vi "DAQmx.AO Max to Range.vi"(11 "AO.Max":dbl) -> (3 "Range":T1)   [LabVIEW 2019, in "DAQmx.lvclass"]
uses:
  DAQmx.lvclass
  typedefs/DAQmx.Config.AO.Range--enum.ctl
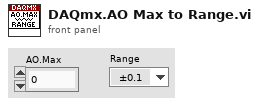
[diagram p1: front panel]
types:
  T1 = typedef "DAQmx.lvclass/DAQmx.Config.AO.Range--enum.ctl" = enum16{"±0.1", "±1.0", "±3.5", "±10.0"}
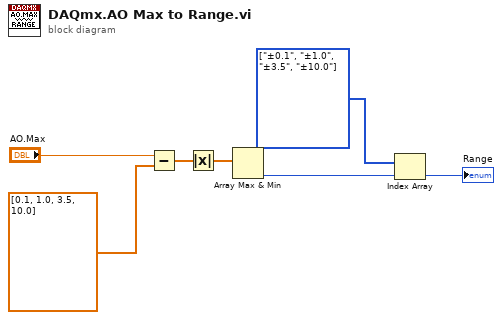
[diagram p0: block diagram]
diagram:
  w3 = T1[] [enum."±0.1", enum."±1.0", enum."±3.5", enum."±10.0"] items=["±0.1", "±1.0", "±3.5", "±10.0"] ("Range")
  n1 = Subtract(x="AO.Max", y=dbl[] [0.1, 1.0, 3.5, 10.0]) -> (x-y=w5:dbl[])
  n2 = Absolute Value(x=w5) -> (abs(x)=w4:dbl[])
  n3 = Array Max & Min(array=w4) -> (min index (indices)=w2:i32)  [unwired: 3 out]
  n4 = Index Array(array=w3, index=w2) -> (element=→"Range":T1)
